vi "Host_Popup_Manager.vi"(8 "error in (no error)":errorcluster={"status"=FALSE, "code"=0, "source"="\"\""}, 10 "run and request IDs":string, 11 "PopupRequest":string) -> (0 "error out":errorcluster={"status"=FALSE, "code"=0, "source"="\"\""}, 2 "status ok":bool, 3 "PopupAck":string)   [LabVIEW 2026]
doc: "INTENT: Show operator instructions and ACK. LOGIC: Display requested text, elapsed-time feedback and options; send ACK only for active request; close on stop/fault."
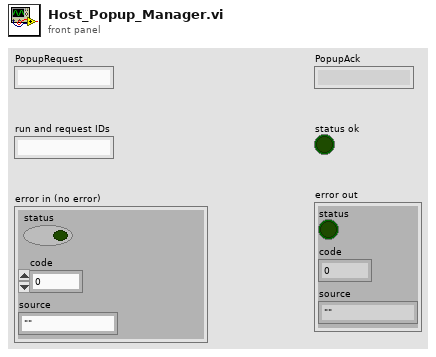
[diagram p1: front panel]
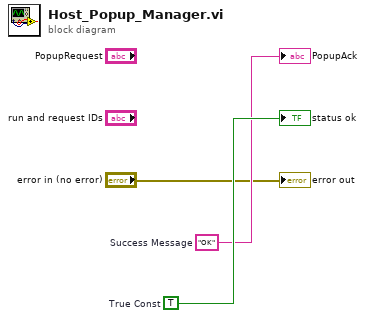
[diagram p0: block diagram]
diagram:
  w3 = TRUE  # True Const
  w2 = "OK"  # Success Message
  "PopupAck" <- w2
  "status ok" <- w3
  "error out" <- "error in (no error)"
